vi "Exemple - Engine Move Object.vi"() -> ()   [LabVIEW 2012]
uses:
  Engine/Move Speed.ctl
  <vilib>/Utility/miscctls.llb/LVPositionTypeDef.ctl
panel:
  in  "Move":bool
  in  "Ball":bool
  in  "Move Speed (Fast)":T1=enum."Fast"
  # "There are three ways to show the UI Engine's position control:\n\nA)  LEFT-CLICK on the control to change its value normally (toggle)\n\nB) Hold down Ctrl key and use LEFT-CLICK anywhere on Front Panel to have the Ball move to the clicked position (at Move Speed)\n\nC) Hold down Shift key and drag the Ball by pressing the LEFT-CLICK button. Release the Ball when you release the button."
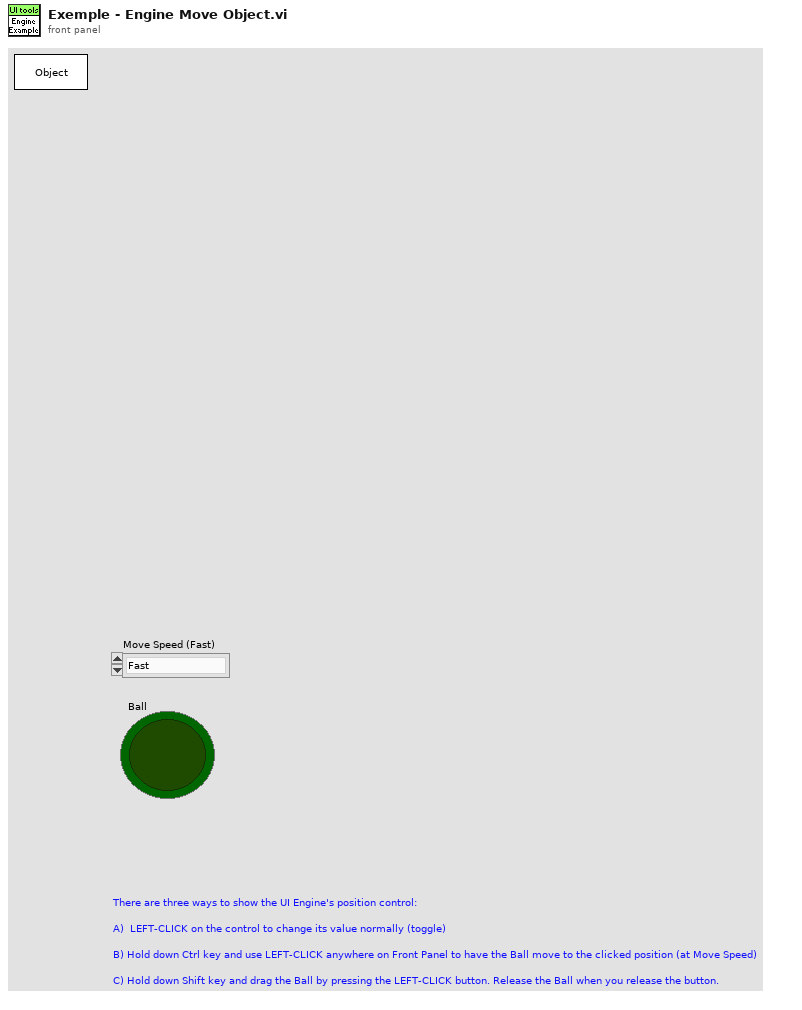
[diagram p1: front panel]
types:
  T1 = typedef "Move Speed.ctl" = enum16{"Normal", "Fast", "Slow", "Instantaneous"}
  T2 = typedef "LVPositionTypeDef.ctl" = cluster{"Left":i32, "Top":i32}
  T3 = enum32{"invalid app kind", "Development System", "Run Time System", "Student Edition", "Embedded LabVIEW", "Evaluation", "Custom"}
  T4 = typedef "LVPoint32TypeDef.ctl" = cluster{"Horizontal":i32, "Vertical":i32}
  T5 = cluster{"Shift":bool, "Ctrl":bool, "Alt":bool, "Cmd":bool, "Opt":bool}
  T6 = typedef "LVBoundsTypeDef.ctl" = cluster{"Width":u32, "Height":u32}
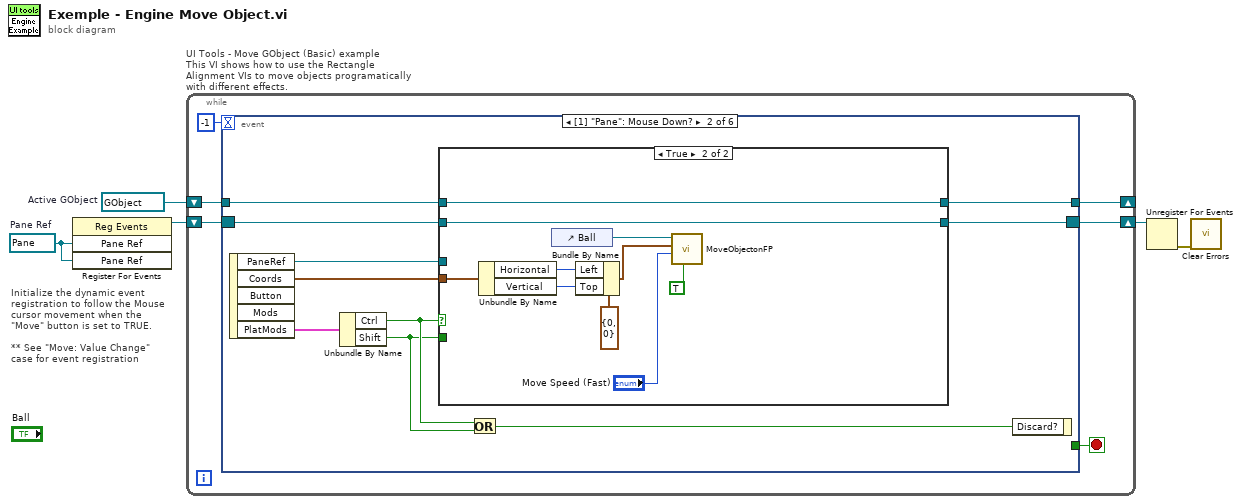
[diagram p0: block diagram]
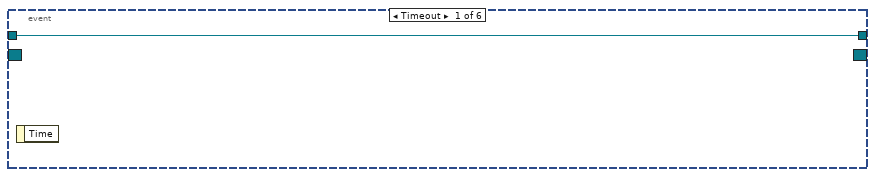
[diagram p2: hidden frame]
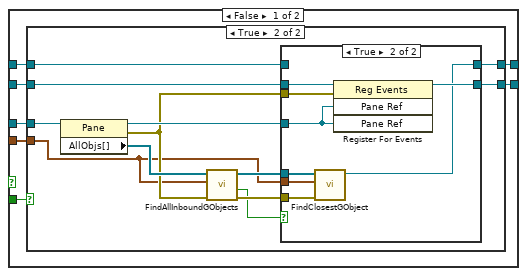
[diagram p3: hidden frame]
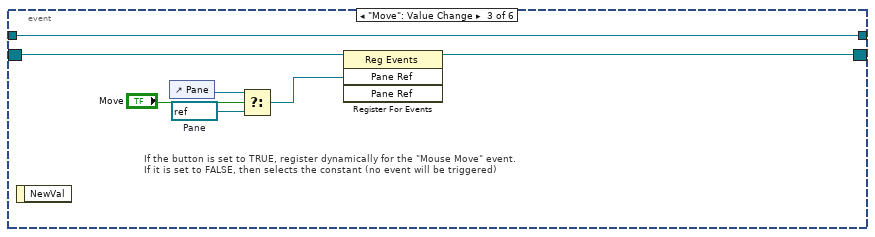
[diagram p6: hidden frame]
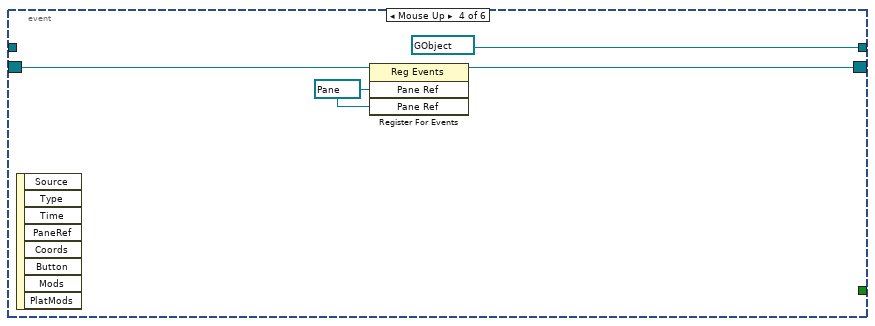
[diagram p7: hidden frame]
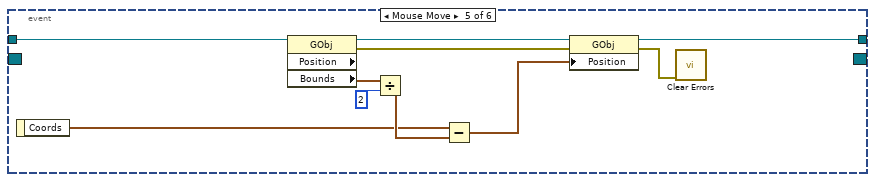
[diagram p8: hidden frame]
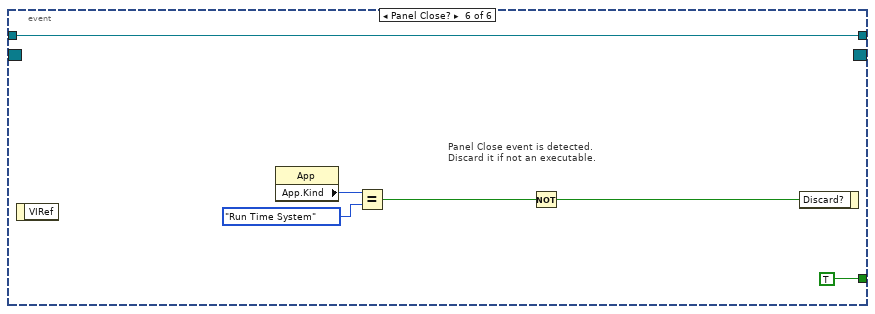
[diagram p9: hidden frame]
diagram:
  w1 = refnum<vi> refnum  # Active GObject
  w2 = refnum<vi> refnum  # Pane Ref
  # "Initialize the dynamic event\nregistration to follow the Mouse\ncursor movement when the\n\"Move\" button is set to TRUE.\n\n** See \"Move: Value Change\"\ncase for event registration"
  n1 = register-events(w2, w2) -> (reference out=w5:refnum<event-registration>)  [unwired: 2 in, 1 out]
  n2 = while "UI Tools - Move GObject (Basic) example\nThis VI shows how to use the Rectangle Alignment VIs to move objects programatically with different effects." {
    shift-right: [w8] -> w3
    shift-left: w5 -> [w9]
    shift-right: [w6] -> _
    shift-left: w1 -> [w7]
    stop <- w10 stop-if-true
    n3 = event shown="[1] \"Pane\": Mouse Down?" {
      selector: w9 -> [_ w17 w69 w73 _ _]
      dyn-events: [_ w16 w67 w72 _ _] -> w8
      timeout: -1 -> [_ _ _ _ _ _]
      tunnel: [_ _ _ _ _ TRUE ("Discard?")] -> w10
      tunnel: w7 -> [w12 w19 w64 _ w76 w85]
      tunnel: [w12 w18 w64 refnum<vi> refnum ("Active GObject") w75 w85] -> w6
      event Timeout {
        n4 = event-data() -> ()  [unwired: 2 out]
      }
      event Mouse Down? {
        n5 = event-data() -> ("PaneRef"=w21:refnum<vi>, "Coords"=w20:T4, "PlatMods"=w22:T5)  [unwired: 3 out]
        n6 = Unbundle By Name(w22) -> ("Ctrl"=w15:bool, "Shift"=w14:bool)
        n7 = case shown="True" w15 {
          tunnel: w19 -> [w25 w63]
          tunnel: [w24 w63] -> w18
          tunnel: w20 -> [w26 w59]
          tunnel: w14 -> [w23 _]
          tunnel: w17 -> [w29 w56]
          tunnel: [w28 w56] -> w16
          tunnel: w21 -> [w27 _]
          frame False {
            n8 = case shown="True" w23 {
              tunnel: w29 -> [w31 w43]
              tunnel: [w31 w42] -> w28
              tunnel: w27 -> [_ w39]
              tunnel: w26 -> [_ w32]
              tunnel: w25 -> [w30 w41]
              tunnel: [w30 w40] -> w24
              frame False {
              }
              frame True {
                n9 = property class="Pane"(reference=w39) -> (reference out=w36:refnum<vi>, error out=w34:errorcluster, "AllObjs[]"=w38:refnum<vi>[])  [unwired: 1 in]
                n10 = call "FindAllInboundGObjects.vi"("error in (no error)"=w34, "Coordinates"=w32, "List of GObjects"=w38) -> ("error out"=w35:errorcluster, "Inbound objects found?"=w33:bool, "Inbound GObjects"=w37:refnum<vi>[])  [unwired: 6 out]
                n11 = case shown="True" w33 {
                  tunnel: w43 -> [w45 w53]
                  tunnel: [w45 w52] -> w42
                  tunnel: w41 -> [w44 _]
                  tunnel: [w44 w46] -> w40
                  tunnel: w37 -> [_ w51]
                  tunnel: w36 -> [_ w50]
                  tunnel: w32 -> [_ w49]
                  tunnel: w35 -> [_ w48]
                  tunnel: w34 -> [_ w47]
                  frame False {
                  }
                  frame True {
                    n12 = call "FindClosestGObject.vi"("error in (no error)"=w48, "Coordinates"=w49, "List of GObjects"=w51) -> ("Closest GObject"=w46:refnum<vi>)  [unwired: 8 out]
                    n13 = register-events(reference=w53, error in=w47, w50, w50) -> (reference out=w52:refnum<event-registration>)  [unwired: 1 out]
                  }
                }
              }
            }
          }
          frame True {
            n14 = Unbundle By Name(w59) -> ("Horizontal"=w57:i32, "Vertical"=w58:i32)
            n15 = control-ref of="Ball"() -> (w55:refnum<vi>)
            n16 = Bundle By Name(cluster=T2 {"Left"=0, "Top"=0} ("Desired Position"), "Left"=w57, "Top"=w58) -> (w60:T2)
            n17 = call "MoveObjectonFP.vi"("Obsolete"=TRUE ("Blocking? (F)"), "Move Speed (Instantaneous)"="Move Speed (Fast)", "Center Position for Object"=w60, "GObject"=w55) -> ()  [unwired: 2 in, 6 out]
          }
        }
        n18 = Or(x=w15, y=w14) -> (x .or. y?=w13:bool)
        n19 = event-data("Discard?"=w13) -> ()  [unwired: 1 in, 1 out]
      }
      event "Move": Value Change {
        w70 = refnum<vi> refnum  # Pane
        # "If the button is set to TRUE, register dynamically for the \"Mouse Move\" event.\nIf it is set to FALSE, then selects the constant (no event will be triggered)"
        n20 = event-data() -> ()  [unwired: 2 out]
        n21 = control-ref of="Pane"() -> (w65:refnum<vi>)
        n22 = Select(t=w65, s="Move", f=w70) -> (s? t:f=w68:refnum<vi>)
        n23 = register-events(reference=w69, w68) -> (reference out=w67:refnum<event-registration>)  [unwired: 2 in, 1 out]
      }
      event Mouse Up {
        w74 = refnum<vi> refnum ("event source")
        n24 = event-data() -> ()  [unwired: 9 out]
        n25 = register-events(reference=w73, w74, w74) -> (reference out=w72:refnum<event-registration>)  [unwired: 1 in, 1 out]
      }
      event Mouse Move {
        n26 = event-data() -> ("Coords"=w77:T4)  [unwired: 1 out]
        n27 = property class="GObj" props=["Position", "Bounds"](reference=w76) -> (reference out=w80:refnum<vi>, error out=w83:errorcluster, "Bounds"=w78:T6)  [unwired: 1 in, 1 out]
        n28 = Divide(x=w78, y=2) -> (x/y=w81:cluster{"Width":dbl, "Height":dbl})
        n29 = Subtract(x=w77, y=w81) -> (x-y=w82:cluster{dbl, dbl})
        n30 = property class="GObj"(reference=w80, error in=w83, "Position"=w82) -> (reference out=w75:refnum<vi>, error out=w84:errorcluster)
        n31 = call <vilib>:"Clear Errors.vi"("error in (no error)"=w84) -> ()  [unwired: 7 out]
      }
      event Panel Close? {
        # "Panel Close event is detected.\nDiscard it if not an executable."
        n32 = event-data() -> ()  [unwired: 2 out]
        n33 = property class="App"() -> ("App.Kind"=w89:T3)  [unwired: 2 in, 2 out]
        n34 = Equal?(x=w89, y=T3."Run Time System" ("Application:Kind")) -> (x = y?=w88:bool)
        n35 = Not(x=w88) -> (.not. x?=w86:bool)
        n36 = event-data("Discard?"=w86) -> ()  [unwired: 1 in, 1 out]
      }
    }
  }
  n37 = Unregister For Events(event registration refnum=w3) -> (error out=w4:errorcluster)  [unwired: 1 in]
  n38 = call <vilib>:"Clear Errors.vi"("error in (no error)"=w4) -> ()  [unwired: 7 out]
